vi "GOOP_LVClass_CreateNewWizard_Invoke.vi"(10 "New Item Parent":T1, 11 "Wizard":u64) -> (3 "Canceled":bool)   [LabVIEW 2020]
uses:
  ClassProviders/Provider_BaseClassInterface/ClassWriter_class/ClassWriter.lvclass
  ClassProviders/Provider_EndevoGOOP300/GOOP300_SubVIs/GOOP300_MethodScopeType.ctl
  SubVIs/GOOP_ClassProviderClassType.ctl
  <resource>/Framework/Providers/API/mxLvNIIM.ctl
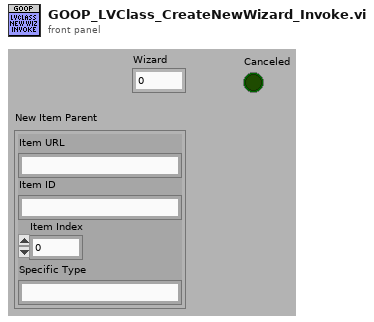
[diagram p1: front panel]
types:
  T1 = typedef "mxLvNIIM.ctl" = cluster{"Item URL":string, "Item ID":string, "Item Index":i32, "Specific Type":string}
  T2 = typedef "GOOP300_MethodScopeType.ctl" = enum16{"Use Parent Folder Scope", "Public", "Protected", "Private", "Community"}
  T3 = typedef "GOOP_ClassProviderClassType.ctl" = enum16{"ClassWriter", "ClassReader"}
  T4 = typedef "ClassWriter.lvclass/InterfacesToImplement.ctl" = cluster{"InterfacePath":path[], "CreateMethods":bool, "MethodsPerInterface(Empty=>All)":cluster{"Methods":string[]}[]}
  T5 = typedef "ClassWriter.lvclass/CreateClassData.ctl" = cluster{"ClassName":string, "ClassFolder":path, "ClassDescription":string, "ClassTemplateOptions":string, "BaseClass(ProjectStringPath or LvClassFilePath)":variant, "ExtraCreateParameters":variant, "FolderSuffix":string, "ParentInterfaces":path[]}
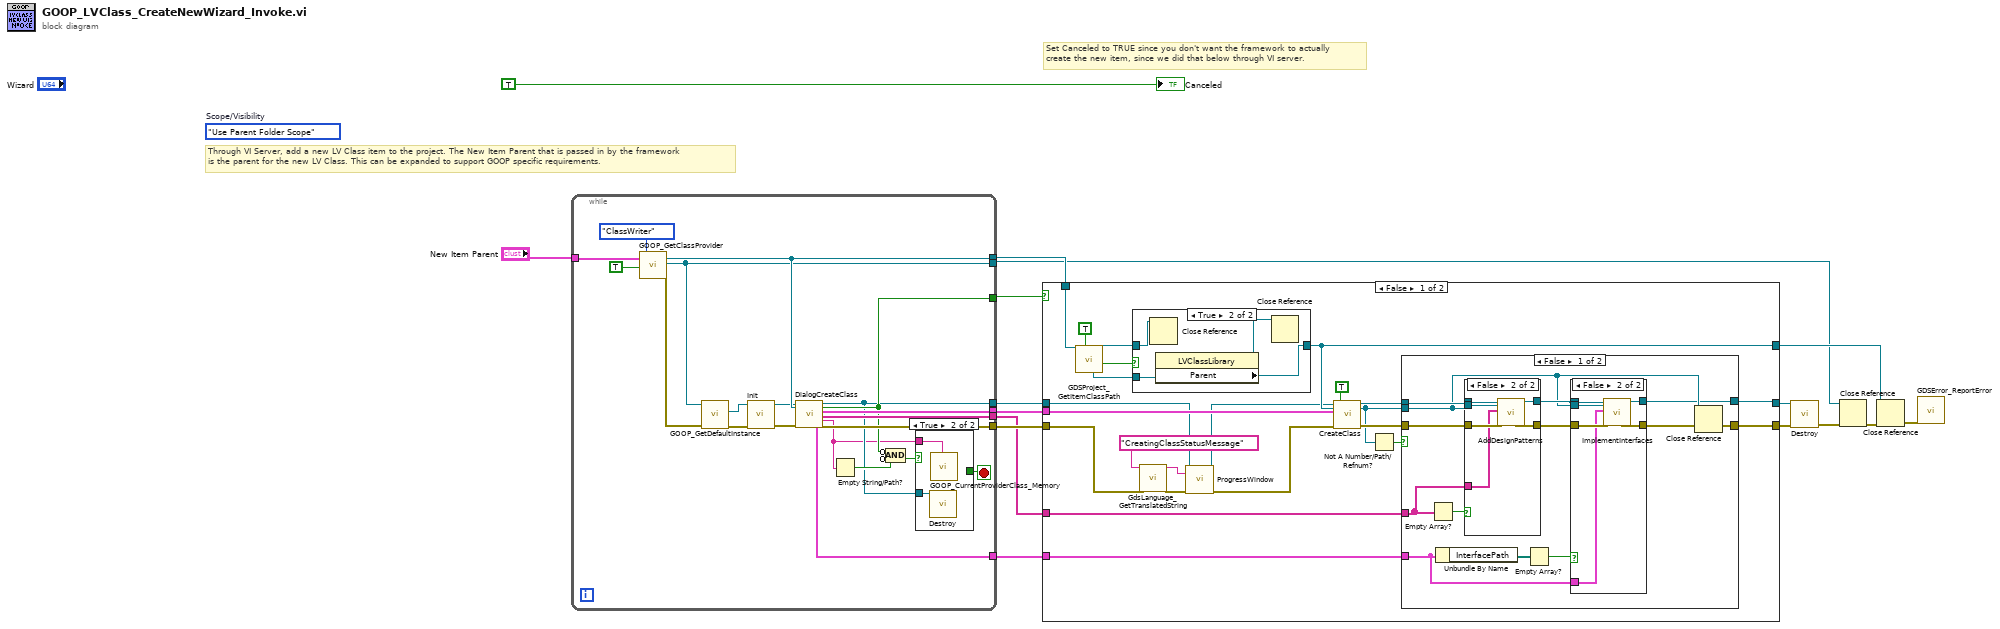
[diagram p0: block diagram]
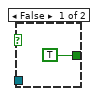
[diagram p2: hidden frame]
diagram:
  (unwired) GOOP300_MethodScopeType."Use Parent Folder Scope"  # Scope/Visibility
  # "Through VI Server, add a new LV Class item to the project. The New Item Parent that is passed in by the framework\nis the parent for the new LV Class. This can be expanded to support GOOP specific requirements."
  # "Set Canceled to TRUE since you don't want the framework to actually\ncreate the new item, since we did that below through VI server."
  n1 = while {
    tunnel: "New Item Parent" -> [w36]
    tunnel: [w19] -> w12
    tunnel: [w35] -> w11
    tunnel: [w34] -> w10
    tunnel: [w32] -> w7
    tunnel: [w27] -> w4
    tunnel: [w24] -> w3
    tunnel: [w23] -> w2
    tunnel: [w17] -> w1
    stop <- w20 stop-if-true
    n2 = call "GOOP_GetClassProvider.vi"("New Item Parent/Object"=w36, "CreateClass"=TRUE, "ProviderClassType"=GOOP_ClassProviderClassType."ClassWriter") -> ("ProjectItem"=w32:refnum<vi>, "LVClass.Open"=w27:refnum<vi>, "error out"=w26:errorcluster)  [unwired: 14 in]
    n3 = call "GOOP_GetDefaultInstance.vi"("error in"=w26, "LVClassIn"=w27) -> ("error out"=w28:errorcluster, "ClassWriter.lvclass"=w25:refnum<class "ClassWriter.lvclass">)  [unwired: 7 in, 1 out]
    n4 = call-dynamic "Init.vi"("ClassWriter in"=w25, "error in (no error)"=w28) -> ("ClassWriter out"=w30:refnum<class "ClassWriter.lvclass">, "error out"=w29:errorcluster)  [unwired: 16 in]
    n5 = call-dynamic "DialogCreateClass.vi"("ClassWriter in"=w30, "ProjectItem Refnum"=w32, "error in (no error)"=w29) -> ("InterfaceToImplement"=w17:T4, "ClassWriter out"=w19:refnum<class "ClassWriter.lvclass">, "Cancelled"=w23:bool, "CreateClassData"=w34:T5, "DesignPatternsToAddAfterCreation"=w24:string[], "ChangeProviderRequested"=w18:string, "error out"=w35:errorcluster)  [unwired: 10 in]
    n6 = Empty String/Path?(string/path=w18) -> (empty?=w22:bool)
    n7 = Compound Arithmetic op=AND(invert w23, invert w22) -> (w21:bool)
    n8 = case shown="True" w21 {
      tunnel: w18 -> [_ w39]
      tunnel: [TRUE _] -> w20
      tunnel: w19 -> [_ w38]
      frame False {
      }
      frame True {
        n9 = call-dynamic "Destroy.vi"("ClassWriter.lvclass"=w38) -> ()  [unwired: 18 in, 1 out]
        n10 = call "GOOP_CurrentProviderClass_Memory.vi"("SetDefaultClassProvider(Ignored if not wired)"=w39) -> ()  [unwired: 12 in, 7 out]
      }
    }
  }
  n11 = case shown="False" w2 {
    tunnel: [w43 w101] -> w15
    tunnel: [w50 w100] -> w14
    tunnel: w12 -> [w53 w101]
    tunnel: w11 -> [w47 w100]
    tunnel: w10 -> [w62 _]
    tunnel: w7 -> [w61 w99]
    tunnel: [w57 w99] -> w6
    tunnel: w3 -> [w46 _]
    tunnel: w1 -> [w40 _]
    frame False {
      n12 = call "GDSProject_GetItemClassPath.vi"("ReturnRefToClass(False)"=TRUE, "ProjectItemRefIn"=w61) -> ("LvCLassFound"=w59:bool, "ProjectItemRefOut"=w58:refnum<vi>, "LvClassRef"=w56:refnum<vi>)  [unwired: 4 in, 3 out]
      n13 = case shown="True" w59 {
        tunnel: w58 -> [w94 w98]
        tunnel: [w94 w96] -> w57
        tunnel: w56 -> [_ w97]
        frame False {
        }
        frame True {
          n14 = Close Reference(reference=w98) -> ()  [unwired: 1 in, 1 out]
          n15 = property class="LVClassLibrary"(reference=w97) -> (reference out=w95:refnum<vi>, "Parent"=w96:refnum<vi>)  [unwired: 1 in, 1 out]
          n16 = Close Reference(reference=w95) -> ()  [unwired: 1 in, 1 out]
        }
      }
      n17 = call "GdsLanguage_GetTranslatedString.vi"("StringID(s)"="CreatingClassStatusMessage" ("Message(Exit)"), "error in (no error)"=w47) -> ("FirstStringOut"=w55:string, "error out"=w48:errorcluster)  [unwired: 14 in, 2 out]
      n18 = call-dynamic "ProgressWindow.vi"("ClassWriter in"=w53, "Message(Exit)"=w55, "error in (no error)"=w48) -> ("ClassWriter out"=w52:refnum<class "ClassWriter.lvclass">, "error out"=w49:errorcluster)  [unwired: 15 in]
      n19 = call-dynamic "CreateClass.vi"("ClassWriter.lvclass"=w52, "ProjectTreePosition(String or Project Item Ref)"=w57, "CreateClassData"=w62, "error in (no error)"=w49, "KeepLvClassRefOpen(False)"=TRUE) -> ("ClassWriter.lvclass"=w45:refnum<class "ClassWriter.lvclass">, "LVClassLibraryRefnum"=w42:refnum<vi>, "error out"=w44:errorcluster)  [unwired: 11 in, 1 out]
      n20 = Not A Number/Path/Refnum?(number/path/refnum=w42) -> (NaN/Path/Refnum?=w41:bool)
      n21 = case shown="False" w41 {
        tunnel: [w75 w93] -> w50
        tunnel: w46 -> [w70 _]
        tunnel: w45 -> [w74 w92]
        tunnel: w44 -> [w73 w93]
        tunnel: [w65 w92] -> w43
        tunnel: w42 -> [w66 _]
        tunnel: w40 -> [w63 _]
        frame False {
          n22 = Empty Array?(array=w70) -> (empty?=w69:bool)
          n23 = Unbundle By Name(w63) -> ("InterfacePath"=w71:path[])
          n24 = case shown="False" w69 {
            tunnel: w74 -> [w85 w91]
            tunnel: w73 -> [w84 w90]
            tunnel: [w84 w89] -> w72
            tunnel: [w85 w88] -> w67
            tunnel: w70 -> [_ w87]
            tunnel: w66 -> [_ w86]
            frame True {
            }
            frame False {
              n25 = call-dynamic "AddDesignPatterns.vi"("ClassWriterNative"=w91, "ClassItemRefIn"=w86, "DesignPatterns"=w87, "error in (no error)"=w90) -> ("ClassWriterNative"=w88:refnum<class "ClassWriter.lvclass">, "error out"=w89:errorcluster)  [unwired: 12 in, 2 out]
            }
          }
          n26 = Empty Array?(array=w71) -> (empty?=w68:bool)
          n27 = case shown="False" w68 {
            tunnel: w67 -> [w77 w83]
            tunnel: w72 -> [w76 w82]
            tunnel: [w76 w81] -> w64
            tunnel: [w77 w80] -> w65
            tunnel: w63 -> [_ w79]
            tunnel: w66 -> [_ w78]
            frame True {
            }
            frame False {
              n28 = call-dynamic "ImplementInterfaces.vi"("ClassWriterNative"=w83, "ClassItemRefIn"=w78, "InterfacesToImplement"=w79, "error in (no error)"=w82) -> ("ClassWriterNative"=w80:refnum<class "ClassWriter.lvclass">, "error out"=w81:errorcluster)  [unwired: 12 in, 2 out]
            }
          }
          n29 = Close Reference(reference=w66, error in (no error)=w64) -> (error out=w75:errorcluster)
        }
        frame True {
        }
      }
    }
    frame True {
    }
  }
  n30 = call-dynamic "Destroy.vi"("ClassWriter.lvclass"=w15, "error in (no error)"=w14) -> ("error out"=w9:errorcluster)  [unwired: 17 in]
  n31 = Close Reference(reference=w4, error in (no error)=w9) -> (error out=w8:errorcluster)
  n32 = Close Reference(reference=w6, error in (no error)=w8) -> (error out=w5:errorcluster)
  n33 = call "GDSError_ReportError.vi"("error in (no error)"=w5) -> ()  [unwired: 18 in, 1 out]
  "Canceled" <- TRUE ("Canceled")
